vi "set Modulation Index Table Type.vi"(8 "error in (no error)":errorcluster, 9 "256QAM Enable":bool, 10 "64QAM Enable":bool, 11 "LTE in":refnum<class "LTE.lvclass">) -> (0 "error out":errorcluster, 3 "LTE out":refnum<class "LTE.lvclass">)   [LabVIEW 2023, in "ANRITSU Call Box.lvlib" / "LTE.lvclass"]
uses:
  LTE.lvclass
  LTE.lvclass/LTE.ctl
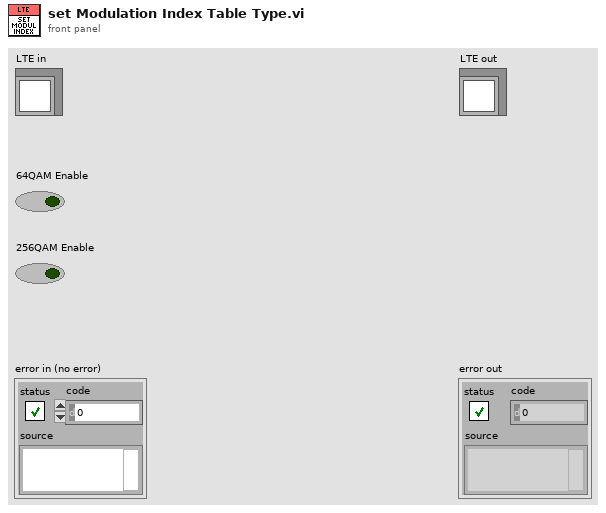
[diagram p1: front panel]
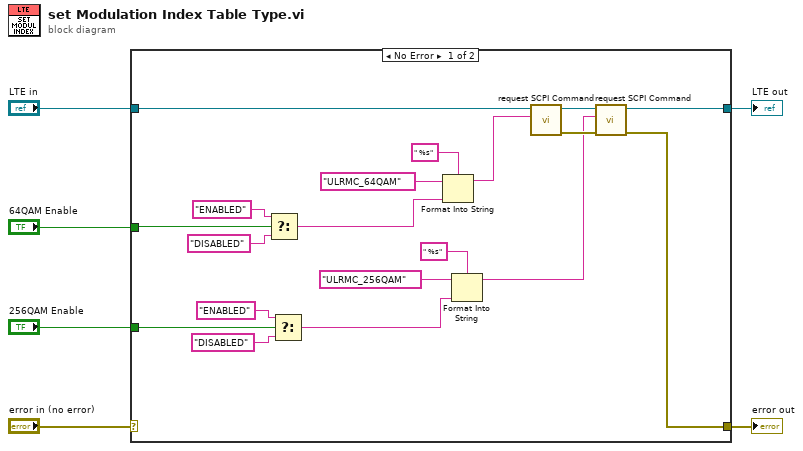
[diagram p0: block diagram]
diagram:
  n1 = case shown="No Error" "error in (no error)" {
    selector: "error in (no error)" -> [_ w27]
    tunnel: [w8 w27] -> w5
    tunnel: [w7 w26] -> w3
    tunnel: "LTE in" -> [w13 w26]
    tunnel: "64QAM Enable" -> [w25 _]
    tunnel: "256QAM Enable" -> [w20 _]
    frame No Error {
      n2 = Select(t="ENABLED", s=w25, f="DISABLED") -> (s? t:f=w17:string)
      n3 = Select(t="ENABLED", s=w20, f="DISABLED") -> (s? t:f=w14:string)
      n4 = Format Into String(format string=" %s", initial string="ULRMC_64QAM", w17) -> (resulting string=w12:string)  [unwired: 1 in, 1 out]
      n5 = Format Into String(format string=" %s", initial string="ULRMC_256QAM", w14) -> (resulting string=w9:string)  [unwired: 1 in, 1 out]
      n6 = call "request SCPI Command.vi"("SCPI Command"=w12, "LTE in"=w13) -> ("error out"=w10:errorcluster, "LTE out"=w11:refnum<class "LTE.lvclass">)  [unwired: 8 in]
      n7 = call "request SCPI Command.vi"("error in (no error)"=w10, "SCPI Command"=w9, "LTE in"=w11) -> ("error out"=w8:errorcluster, "LTE out"=w7:refnum<class "LTE.lvclass">)  [unwired: 7 in]
    }
    frame Error {
    }
  }
  "error out" <- w5
  "LTE out" <- w3
